vi "User in Group.vi"(4 "error in (no error)":errorcluster, 5 "Group Name":string, 6 "LoginName":string, 7 "EasyUserManager in":refnum<class "EasyUserManager.lvclass">) -> (0 "error out":errorcluster, 2 "User in Group":bool, 3 "EasyUserManager out":refnum<class "EasyUserManager.lvclass">)   [LabVIEW 2024, in "EasyUserManager.lvclass"]
doc: "Check if the user specified by <B>LoginName</B> is a member of the group specified by <B>Group Name</B>."
uses:
  EasyUserManager.lvclass
  EasyUserManager.lvclass/EasyUserManager.ctl
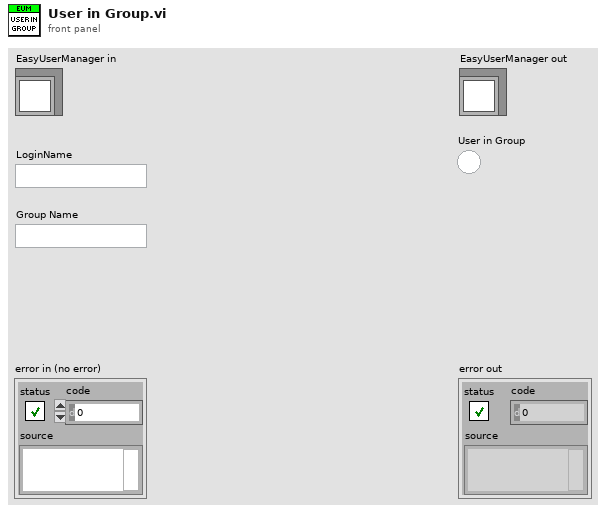
[diagram p1: front panel]
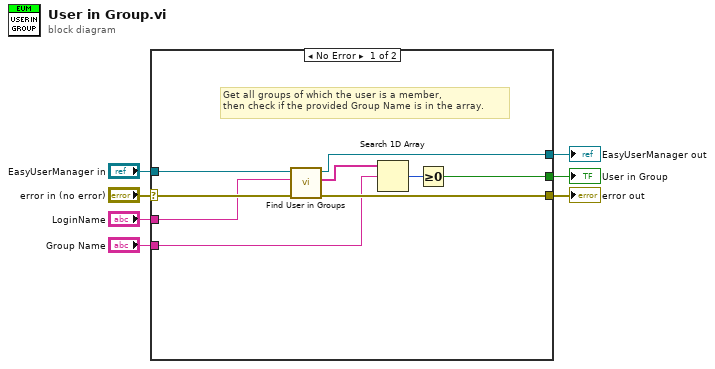
[diagram p0: block diagram]
diagram:
  n1 = case shown="No Error" "error in (no error)" {
    selector: "error in (no error)" -> [w11 w18]
    tunnel: [w13 w18] -> w6
    tunnel: [w15 w17] -> w4
    tunnel: "EasyUserManager in" -> [w14 w17]
    tunnel: "LoginName" -> [w10 _]
    tunnel: "Group Name" -> [w9 _]
    tunnel: [w8 _] -> w1
    frame No Error {
      # "Get all groups of which the user is a member,\nthen check if the provided Group Name is in the array."
      n2 = call "Find User in Groups.vi"("error in (no error)"=w11, "LoginName"=w10, "EasyUserManager in"=w14) -> ("error out"=w13:errorcluster, "Groups"=w16:string[], "EasyUserManager out"=w15:refnum<class "EasyUserManager.lvclass">)  [unwired: 1 in, 1 out]
      n3 = Search 1D Array(1D array=w16, element=w9) -> (index of element=w12:i32)  [unwired: 1 in]
      n4 = Greater Or Equal To 0?(x=w12) -> (x >= 0?=w8:bool)
    }
    frame Error {
      # "Pass error and do nothing"
    }
  }
  "error out" <- w6
  "EasyUserManager out" <- w4
  "User in Group" <- w1
